vi "Add to Query.vi"(8 "error in (no error)":errorcluster, 9 "value":string, 10 "key":string, 11 "URI in":refnum<class "URI.lvclass">) -> (0 "error out":errorcluster, 3 "URI out":refnum<class "URI.lvclass">)   [LabVIEW 2013, in "openURI.lvlib" / "URI.lvclass"]
uses:
  URI.lvclass
  URI.lvclass/URI.ctl
  components/query/URI-Component.Query.lvclass/URI-Component.Query.ctl
  components/query/URI-Component.Query.lvclass
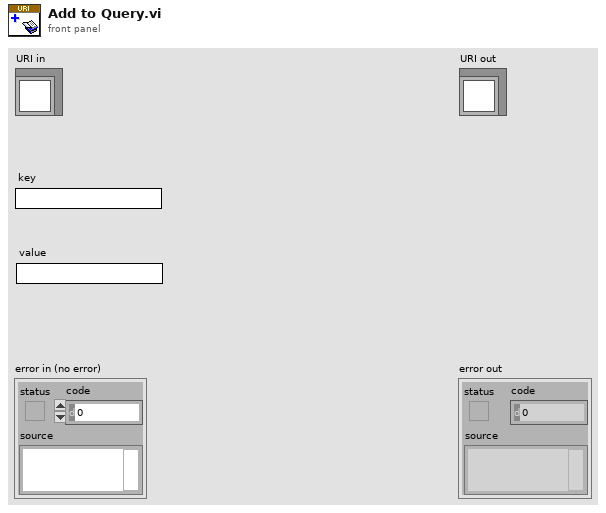
[diagram p1: front panel]
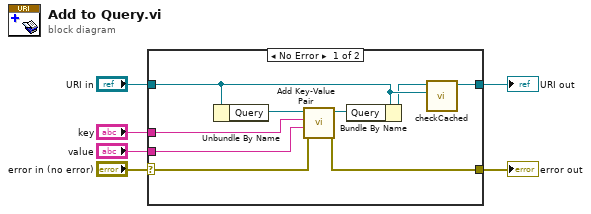
[diagram p0: block diagram]
diagram:
  n1 = case shown="No Error" "error in (no error)" {
    selector: "error in (no error)" -> [w11 w17]
    tunnel: [w10 w17] -> w5
    tunnel: [w7 w16] -> w3
    tunnel: "URI in" -> [w9 w16]
    tunnel: "key" -> [w13 _]
    tunnel: "value" -> [w12 _]
    frame No Error {
      n2 = Unbundle By Name(w9) -> ("Query"=w15:refnum<class "URI-Component.Query.lvclass">)
      n3 = call "Add Key-Value Pair.vi"("error in (no error)"=w11, "value"=w12, "key"=w13, "URI-Component.Query in"=w15) -> ("error out"=w10:errorcluster, "URI-Component.Query"=w14:refnum<class "URI-Component.Query.lvclass">)  [unwired: 6 in]
      n4 = Bundle By Name(cluster=w9, "Query"=w14) -> (w8:refnum<class "URI.lvclass">)
      n5 = call "checkCached.vi"("Old"=w9, "New URI"=w8) -> ("URI"=w7:refnum<class "URI.lvclass">)  [unwired: 9 in]
    }
    frame Error {
    }
  }
  "error out" <- w5
  "URI out" <- w3
